vi "Init Main Panels.vi"(8 "error in (no error)":errorcluster, 11 "picoG in":refnum<class "picoG.lvclass">) -> (0 "error out":errorcluster, 3 "picoG out":refnum<class "picoG.lvclass">)   [LabVIEW 2020, in "PicoG-App.lvlib" / "picoG.lvclass"]
uses:
  picoG.lvclass
  GettingStarted/GettingStarted.lvclass
  C:/Program Files (x86)/National Instruments/LabVIEW 2020/vi.lib/IlluminatedG/IG OOPanel/OOPanel/Panel/Panel.lvclass
  AppDetailPanel/AppDetailPanel.lvclass
  PlatformConfigPanel/PlatformConfigPanel.lvclass
  DeviceDetailPanel/DeviceDetailPanel.lvclass
  picoG.lvclass/picoG.ctl
  <vilib>/IlluminatedG/IG OOPanel/OOPanel/Manager/Manager.lvclass
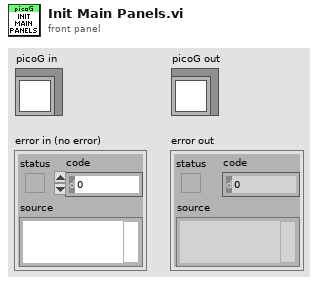
[diagram p1: front panel]
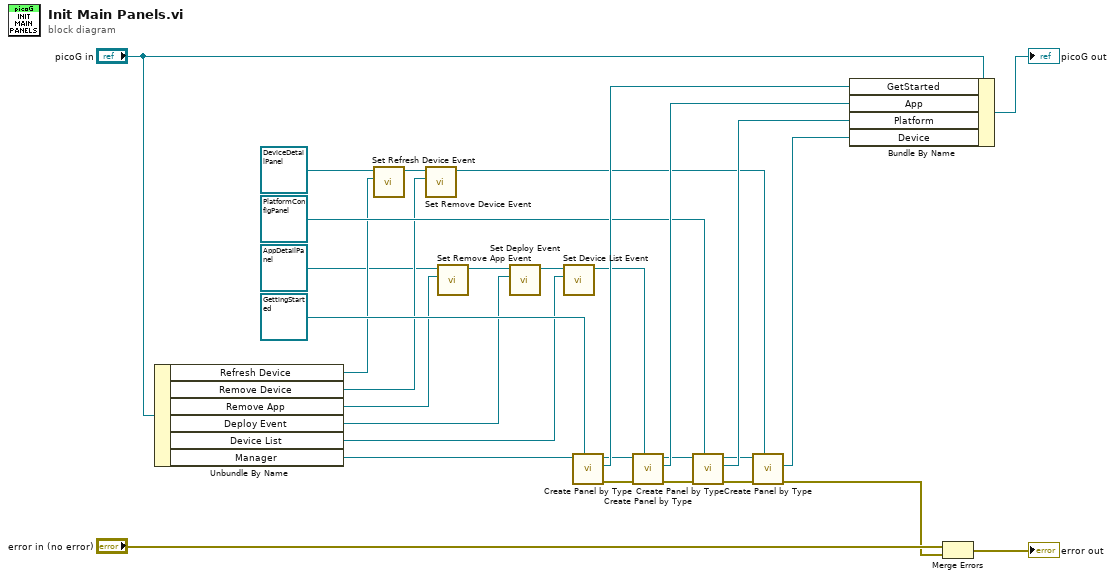
[diagram p0: block diagram]
diagram:
  n1 = Unbundle By Name("picoG in") -> ("Refresh Device"=w4:refnum<user-event>, "Remove Device"=w8:refnum<user-event>, "Remove App"=w1:refnum<user-event>, "Deploy Event"=w9:refnum<user-event>, "Device List"=w12:refnum<user-event>, "Manager"=w27:refnum<class "Manager.lvclass">)
  n2 = call "Set Refresh Device Event.vi"("Refresh Device"=w4, "DeviceDetailPanel in"=refnum<class "DeviceDetailPanel.lvclass"> refnum ("PicoG-App.lvlib:DeviceDetailPanel.lvclass")) -> ("DeviceDetailPanel out"=w6:refnum<class "DeviceDetailPanel.lvclass">)  [unwired: 8 in, 1 out]
  n3 = call "Set Remove Device Event.vi"("Remove Device"=w8, "DeviceDetailPanel in"=w6) -> ("DeviceDetailPanel out"=w7:refnum<class "DeviceDetailPanel.lvclass">)  [unwired: 8 in, 1 out]
  n4 = call "Set Remove App Event.vi"("Remove App"=w1, "AppDetailPanel in"=refnum<class "AppDetailPanel.lvclass"> refnum ("PicoG-App.lvlib:AppDetailPanel.lvclass")) -> ("AppDetailPanel out"=w3:refnum<class "AppDetailPanel.lvclass">)  [unwired: 8 in, 1 out]
  n5 = call "Set Deploy Event.vi"("Deploy Event"=w9, "AppDetailPanel in"=w3) -> ("AppDetailPanel out"=w10:refnum<class "AppDetailPanel.lvclass">)  [unwired: 8 in, 1 out]
  n6 = call "Set Device List Event.vi"("Device List"=w12, "AppDetailPanel in"=w10) -> ("AppDetailPanel out"=w11:refnum<class "AppDetailPanel.lvclass">)  [unwired: 8 in, 1 out]
  n7 = call <vilib>:"Create Panel by Type.vi"("Panel Type"=refnum<class "GettingStarted.lvclass"> refnum ("PicoG-App.lvlib:GettingStarted.lvclass"), "Manager in"=w27) -> ("error out"=w22:errorcluster, "Panel"=w25:refnum<class "GettingStarted.lvclass">, "Manager out"=w24:refnum<class "Manager.lvclass">)  [unwired: 7 in]
  n8 = call <vilib>:"Create Panel by Type.vi"("Panel Type"=w11, "error in (no error)"=w22, "Manager in"=w24) -> ("error out"=w20:errorcluster, "Panel"=w23:refnum<class "AppDetailPanel.lvclass">, "Manager out"=w19:refnum<class "Manager.lvclass">)  [unwired: 6 in]
  n9 = call <vilib>:"Create Panel by Type.vi"("Panel Type"=refnum<class "PlatformConfigPanel.lvclass"> refnum ("PicoG-App.lvlib:PlatformConfigPanel.lvclass"), "error in (no error)"=w20, "Manager in"=w19) -> ("error out"=w15:errorcluster, "Panel"=w17:refnum<class "PlatformConfigPanel.lvclass">, "Manager out"=w16:refnum<class "Manager.lvclass">)  [unwired: 6 in]
  n10 = call <vilib>:"Create Panel by Type.vi"("Panel Type"=w7, "error in (no error)"=w15, "Manager in"=w16) -> ("error out"=w14:errorcluster, "Panel"=w13:refnum<class "DeviceDetailPanel.lvclass">)  [unwired: 6 in, 1 out]
  n11 = Bundle By Name(cluster="picoG in", "GetStarted"=w25, "App"=w23, "Platform"=w17, "Device"=w13) -> (→"picoG out":refnum<class "picoG.lvclass">)
  n12 = Merge Errors("error in (no error)", w14) -> (→"error out":errorcluster)
